vi "DSS-test-saltwater-perm_from_freq.vi"(8 "error in":errorcluster) -> (0 "error out":errorcluster)   [LabVIEW 2020, in "DSS-Tests.lvlib"]
doc: "Caraya test of RDC-saltwater-generate_perm_from_freq: a 300 MHz to 6 GHz sweep (10 MHz steps) at 10, 22.5, 25, 35 and 40 C and four frequencies at 22.5 C, each checked against its golden file."
uses:
  DSS-Tests.lvlib
  <vilib>/addons/_JKI Toolkits/Caraya/classes/Test/Test.lvclass
  <vilib>/addons/_JKI Toolkits/Caraya/classes/Assert/Assert.lvclass
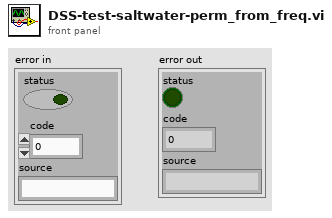
[diagram p1: front panel]
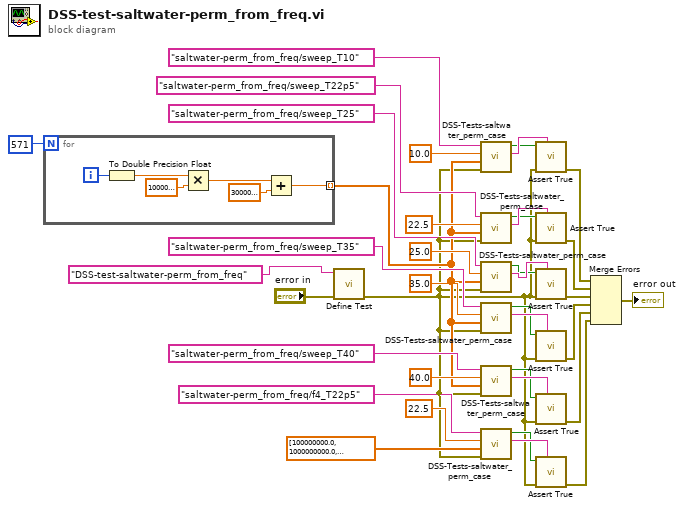
[diagram p0: block diagram]
diagram:
  n1 = for {
    N: 571 ("N") -> [_]
    tunnel: [w43] -> w5 mode=indexing
    i -> [w38]
    n2 = To Double Precision Float(number=w38) -> (double precision float=w39:dbl)
    n3 = Multiply(x=w39, y=10000000.0 ("step")) -> (x*y=w42:dbl)
    n4 = Add(x=w42, y=300000000.0 ("start")) -> (x+y=w43:dbl)
  }
  n5 = call <vilib>:"Define Test.vi"("error in (no error)"="error in", "Label (VI Title)"="DSS-test-saltwater-perm_from_freq") -> ("error out"=w3:errorcluster)  [unwired: 8 in, 1 out]
  n6 = call "DSS-Tests-saltwater_perm_case.vi"("error in"=w3, "frequency"=w5, "temperature"=10.0, "golden name"="saltwater-perm_from_freq/sweep_T10") -> ("message"=w10:string, "pass"=w9:bool)  [unwired: 5 in, 1 out]
  n7 = call "DSS-Tests-saltwater_perm_case.vi"("error in"=w3, "frequency"=w5, "temperature"=22.5, "golden name"="saltwater-perm_from_freq/sweep_T22p5") -> ("message"=w15:string, "pass"=w14:bool)  [unwired: 5 in, 1 out]
  n8 = call "DSS-Tests-saltwater_perm_case.vi"("error in"=w3, "frequency"=w5, "temperature"=25.0, "golden name"="saltwater-perm_from_freq/sweep_T25") -> ("message"=w20:string, "pass"=w19:bool)  [unwired: 5 in, 1 out]
  n9 = call "DSS-Tests-saltwater_perm_case.vi"("error in"=w3, "frequency"=w5, "temperature"=35.0, "golden name"="saltwater-perm_from_freq/sweep_T35") -> ("message"=w25:string, "pass"=w24:bool)  [unwired: 5 in, 1 out]
  n10 = call "DSS-Tests-saltwater_perm_case.vi"("error in"=w3, "frequency"=w5, "temperature"=40.0, "golden name"="saltwater-perm_from_freq/sweep_T40") -> ("message"=w30:string, "pass"=w29:bool)  [unwired: 5 in, 1 out]
  n11 = call "DSS-Tests-saltwater_perm_case.vi"("error in"=w3, "frequency"=dbl[] [100000000.0, 1000000000.0, 3000000000.0, 6000000000.0] ("frequency f4"), "temperature"=22.5, "golden name"="saltwater-perm_from_freq/f4_T22p5") -> ("message"=w35:string, "pass"=w34:bool)  [unwired: 5 in, 1 out]
  n12 = call <vilib>:"Assert True.vi"("Label"=w10, "error in (no error)"=w3, "True?"=w9) -> ("error out"=w11:errorcluster)  [unwired: 7 in, 1 out]
  n13 = call <vilib>:"Assert True.vi"("Label"=w15, "error in (no error)"=w3, "True?"=w14) -> ("error out"=w16:errorcluster)  [unwired: 7 in, 1 out]
  n14 = call <vilib>:"Assert True.vi"("Label"=w20, "error in (no error)"=w3, "True?"=w19) -> ("error out"=w21:errorcluster)  [unwired: 7 in, 1 out]
  n15 = call <vilib>:"Assert True.vi"("Label"=w25, "error in (no error)"=w3, "True?"=w24) -> ("error out"=w26:errorcluster)  [unwired: 7 in, 1 out]
  n16 = call <vilib>:"Assert True.vi"("Label"=w30, "error in (no error)"=w3, "True?"=w29) -> ("error out"=w31:errorcluster)  [unwired: 7 in, 1 out]
  n17 = call <vilib>:"Assert True.vi"("Label"=w35, "error in (no error)"=w3, "True?"=w34) -> ("error out"=w36:errorcluster)  [unwired: 7 in, 1 out]
  n18 = Merge Errors(w11, w16, w21, w26, w31, w36) -> (→"error out":errorcluster)
